vi "Test Build ATM Message.vi"() -> ()   [LabVIEW 2026]
doc: "Caraya unit test for Build ATM Message.vi, generated by lvai_generate_test.\n\nOne static subVI call per case. Every assertion takes its error in from Define Test rather than from the assertion before it, so a failing case cannot stop a later one - chaining them silently loses cases, measured.\n\nThe error cluster carries the FIRST failure only. Read the JUnit report for all of them."
uses:
  <vilib>/addons/_JKI Toolkits/Caraya/classes/Test/Test.lvclass
  <vilib>/addons/_JKI Toolkits/Caraya/classes/Assert/Assert.lvclass
panel:
  out "error out":errorcluster
  in  "error in":errorcluster
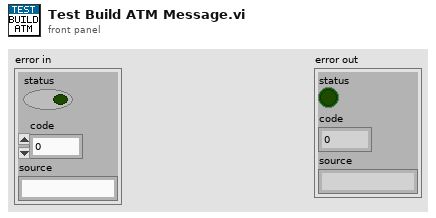
[diagram p1: front panel]
types:
  T1 = cluster{"Account Number":string, "First Name":string, "Last Name":string, "Balance":dbl}
  T2 = enum16{"Welcome", "Main Menu", "Account Verification Failed", "Session Terminate", "Deposit", "Deposit Complete", "Withdrawal", "Withdrawal Complete", "Withdrawal Failed", "Balance Inquiry"}
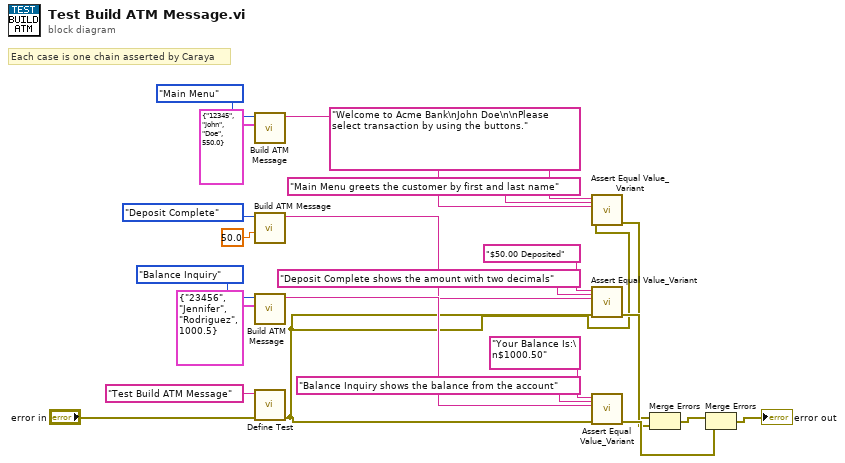
[diagram p0: block diagram]
diagram:
  # "Each case is one chain asserted by Caraya"
  n1 = call "Build ATM Message.vi"("Account"=T1 {"Account Number"="12345", "First Name"="John", "Last Name"="Doe", "Balance"=550.0}, "Message Type"=T2."Main Menu") -> ("ATM Message"=w6:string)  [unwired: 8 in, 1 out]
  n2 = call "Build ATM Message.vi"("Amount"=50.0, "Message Type"=T2."Deposit Complete") -> ("ATM Message"=w12:string)  [unwired: 8 in, 1 out]
  n3 = call "Build ATM Message.vi"("Account"=T1 {"Account Number"="23456", "First Name"="Jennifer", "Last Name"="Rodriguez", "Balance"=1000.5}, "Message Type"=T2."Balance Inquiry") -> ("ATM Message"=w18:string)  [unwired: 8 in, 1 out]
  n4 = call <vilib>:"Define Test.vi"("error in (no error)"="error in", "Label (VI Title)"="Test Build ATM Message") -> ("error out"=w3:errorcluster)  [unwired: 8 in, 1 out]
  n5 = call <vilib>:"Assert Equal Value_Variant.vi"("Label"="Main Menu greets the customer by first and last name", "error in (no error)"=w3, "Actual"=w6, "Expected"="Welcome to Acme Bank\nJohn Doe\n\nPlease select transaction by using the buttons." ("expected 1")) -> ("error out"=w9:errorcluster)  [unwired: 6 in, 1 out]
  n6 = call <vilib>:"Assert Equal Value_Variant.vi"("Label"="Deposit Complete shows the amount with two decimals", "error in (no error)"=w3, "Actual"=w12, "Expected"="$50.00 Deposited" ("expected 2")) -> ("error out"=w15:errorcluster)  [unwired: 6 in, 1 out]
  n7 = call <vilib>:"Assert Equal Value_Variant.vi"("Label"="Balance Inquiry shows the balance from the account", "error in (no error)"=w3, "Actual"=w18, "Expected"="Your Balance Is:\n$1000.50" ("expected 3")) -> ("error out"=w21:errorcluster)  [unwired: 6 in, 1 out]
  n8 = Merge Errors(w9, w15) -> (w22:errorcluster)
  n9 = Merge Errors(w22, w21) -> (→"error out":errorcluster)
